vi "Create Job VI from Template.vi"() -> ()   [LabVIEW 2013]
uses:
  JobCreatorData -- cluster.ctl
panel:
  in  "Cron Job Templates":i32(listbox)
  in  "Instantiate Job":bool
  # "Select a Cron Job Template for instantiation"
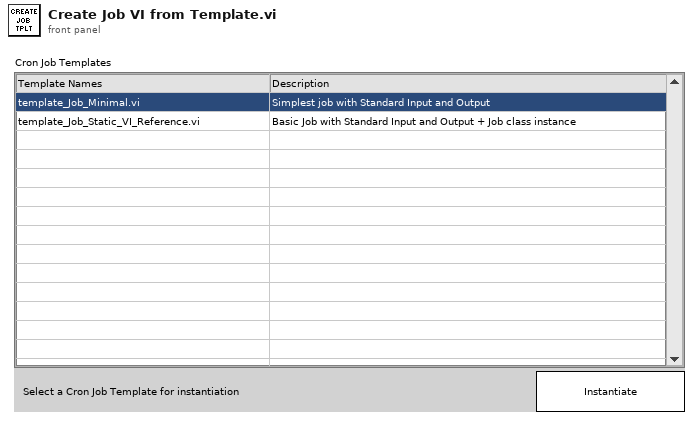
[diagram p1: front panel]
types:
  T1 = enum16{"Initialize", "Discover Template", "Idle", "Create Template", "Exit"}
  T2 = cluster{"App Instance":refnum<vi>, "Active Project":refnum<vi>, "templates":variant, "Cron Folder":path}
  T3 = enum8{"Enabled", "Disabled", "Disabled and Grayed Out"}
  T4 = typedef "JobCreatorData -- cluster.ctl" = cluster{"Path":path, "Name":string, "Description":string}
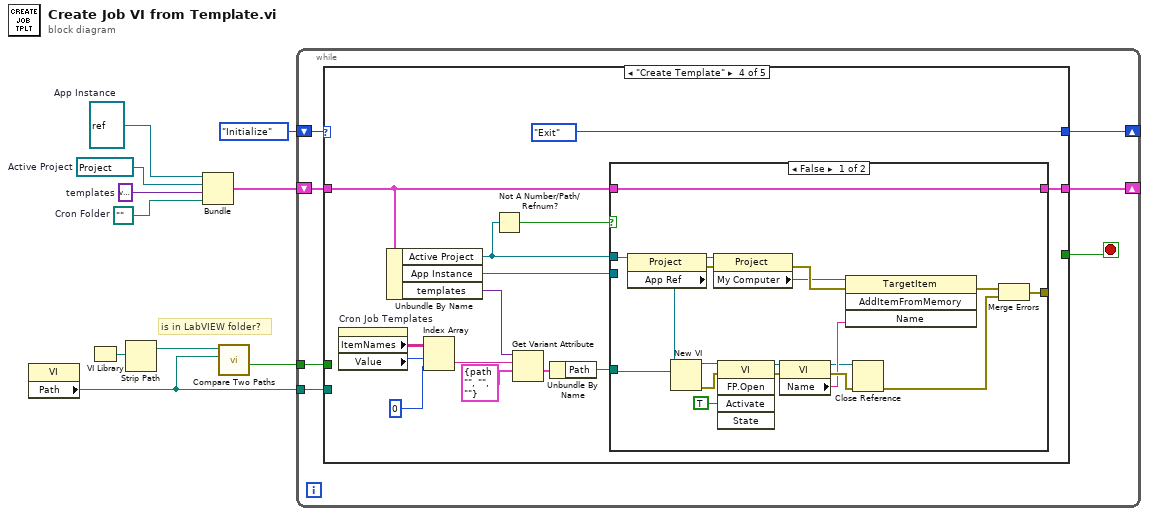
[diagram p0: block diagram]
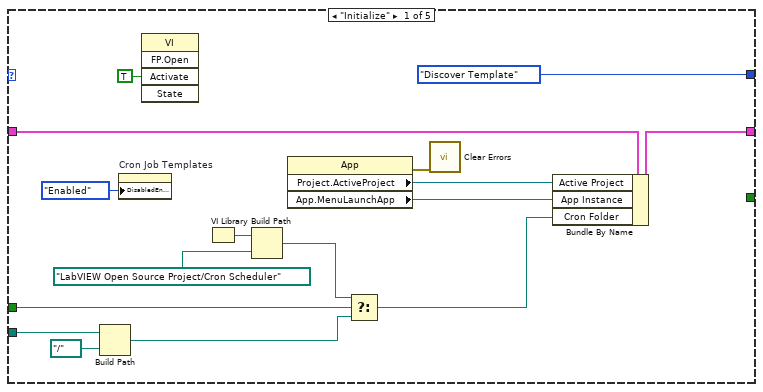
[diagram p2: hidden frame]
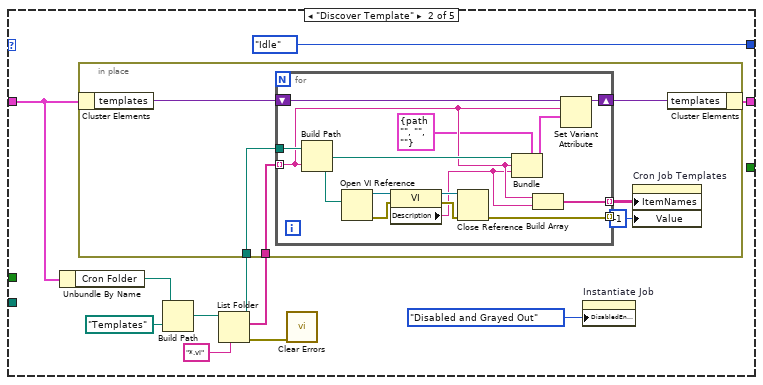
[diagram p3: hidden frame]
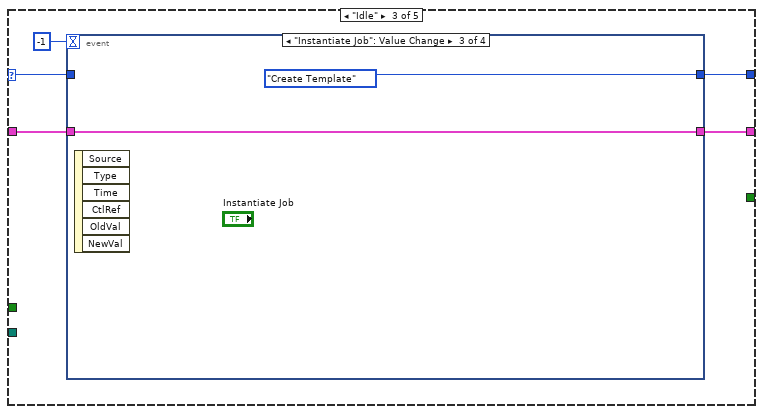
[diagram p4: hidden frame]
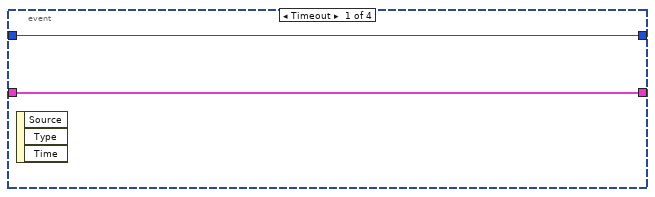
[diagram p5: hidden frame]
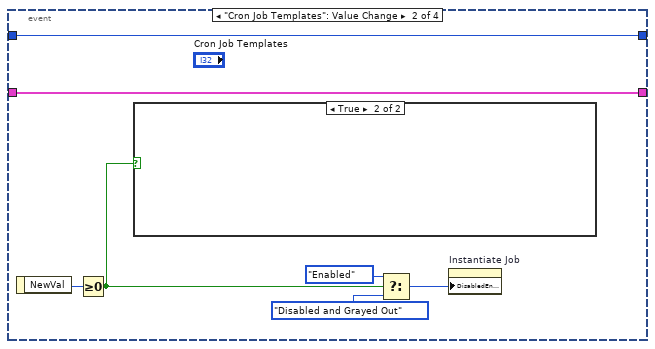
[diagram p6: hidden frame]
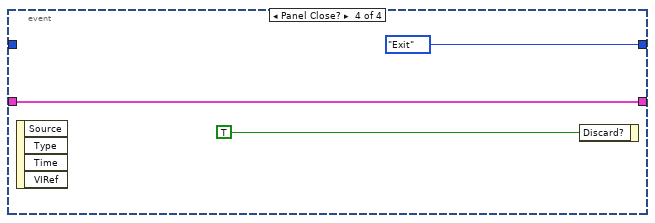
[diagram p8: hidden frame]
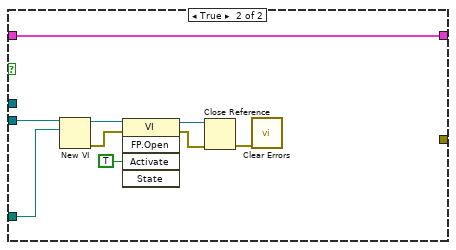
[diagram p9: hidden frame]
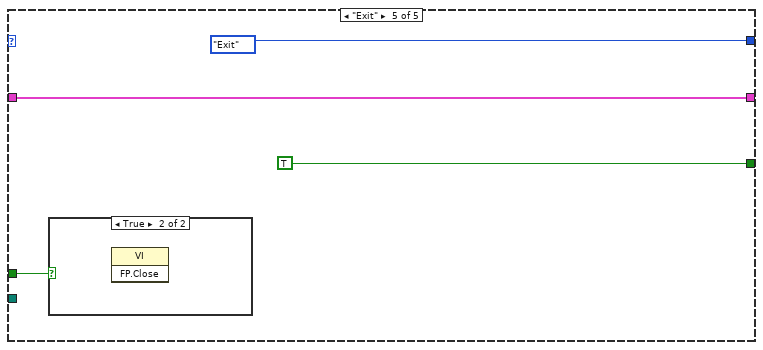
[diagram p10: hidden frame]
diagram:
  w9 = path ""  # Cron Folder
  w8 = variant  # templates
  w7 = refnum<vi> refnum  # App Instance
  w5 = refnum<vi> refnum  # Active Project
  # "is in LabVIEW folder?"
  n1 = property class="VI"() -> ("Path"=w2:path)  [unwired: 2 in, 2 out]
  n2 = VI Library() -> (path=w3:path)
  n3 = Strip Path(path=w3) -> (stripped path=w4:path)  [unwired: 1 out]
  n4 = Bundle("App Instance"=w7, "Active Project"=w5, "templates"=w8, "Cron Folder"=w9) -> (w6:T2)  [unwired: 1 in]
  n5 = call <vilib>:"Compare Two Paths.vi"("Path 2"=w2, "Path 1"=w4) -> ("Path 2 Relative to Path 1?"=w1:bool)  [unwired: 6 in, 3 out]
  n6 = while {
    shift-right: [w16] -> _
    shift-left: T1."Initialize" -> [w17]
    shift-right: [w14] -> _
    shift-left: w6 -> [w15]
    tunnel: w2 -> [w12]
    tunnel: w1 -> [w11]
    stop <- w13 stop-if-true
    n7 = case shown="\"Create Template\"" w17 {
      selector: w17 -> [_ _ w65 _ _]
      tunnel: [T1."Discover Template" T1."Idle" w68 T1."Exit" T1."Exit"] -> w16
      tunnel: w15 -> [w31 w41 w67 w88 w128]
      tunnel: [w32 w43 w66 w87 w128] -> w14
      tunnel: [_ _ _ _ TRUE] -> w13
      tunnel: w12 -> [w19 _ _ _ _]
      tunnel: w11 -> [w18 _ _ _ w126]
      frame "Initialize" {
        n8 = Build Path(base path=w19, name or relative path=path "../.." ("VI Path")) -> (appended path=w27:path)
        n9 = property on="Cron Job Templates" class="MCListbox (strict)"("DisabledEnum"=T3."Enabled" ("Disabled")) -> ()  [unwired: 2 in, 2 out]
        n10 = invoke class="VI" method="FP.Open"("Activate"=TRUE ("Activate?")) -> ()  [unwired: 4 in, 5 out]
        n11 = VI Library() -> (path=w20:path)
        n12 = Build Path(base path=w20, name or relative path=path "LabVIEW Open Source Project/Cron Scheduler" ("VI Path")) -> (appended path=w23:path)
        n13 = property class="App"() -> (error out=w30:errorcluster, "Project.ActiveProject"=w26:refnum<vi>, "App.MenuLaunchApp"=w29:refnum<vi>)  [unwired: 2 in, 1 out]
        n14 = Select(t=w23, s=w18, f=w27) -> (s? t:f=w24:path)
        n15 = call <vilib>:"Clear Errors.vi"("error in (no error)"=w30) -> ()  [unwired: 6 in, 1 out]
        n16 = Bundle By Name(cluster=w31, "Active Project"=w26, "App Instance"=w29, "Cron Folder"=w24) -> (w32:T2)
      }
      frame "Discover Template" {
        n17 = Unbundle By Name(w41) -> ("Cron Folder"=w40:path)
        n18 = Build Path(base path=w40, name or relative path=path "Templates" ("VI Path")) -> (appended path=w39:path)
        n19 = List Folder(path=w39, pattern="*.vi") -> (path out=w36:path, filenames=w37:string[], error out=w35:errorcluster)  [unwired: 2 in, 1 out]
        n20 = in-place {
          in-place-border: w37 -> [w48]
          in-place-border: w36 -> [w47]
          n21 = in-place-cluster #1(w41) -> ("templates"=w50:variant)
          n22 = for {
            tunnel: w48 -> [w54] mode=indexing
            tunnel: w47 -> [w62]
            tunnel: [w57] -> _ mode=indexing
            tunnel: [w52] -> w46 mode=indexing
            shift-right: [w63] -> w49
            shift-left: w50 -> [w64]
            n23 = Build Path(base path=w62, name or relative path=w54) -> (appended path=w60:path)
            n24 = Open VI Reference(vi path=w60) -> (vi reference=w59:refnum<vi>, error out=w56:errorcluster)  [unwired: 5 in]
            n25 = property class="VI"(reference=w59, error in=w56) -> (reference out=w58:refnum<vi>, error out=w55:errorcluster, "Description"=w53:string)
            n26 = Close Reference(reference=w58, error in (no error)=w55) -> (error out=w57:errorcluster)
            n27 = Bundle(cluster=T4 {"Path"=path "", "Name"="", "Description"=""} ("Job Creator Data"), "Path"=w60, "Name"=w54, "Description"=w53) -> (w61:T4)
            n28 = Build Array(w54, w53) -> (w52:string[])
            n29 = Set Variant Attribute(Variant=w64, name=w54, value=w61) -> (Variant out=w63:variant)  [unwired: 1 in, 2 out]
          }
          n30 = property on="Cron Job Templates" class="MCListbox (strict)"("ItemNames"=w46, "Value"=-1 ("Cron Job Templates")) -> ()  [unwired: 2 in, 2 out]
          n31 = in-place-cluster #1("templates"=w49) -> (w43:T2)
        }
        n32 = call <vilib>:"Clear Errors.vi"("error in (no error)"=w35) -> ()  [unwired: 6 in, 1 out]
        n33 = property on="Instantiate Job" class="Bool"("DisabledEnum"=T3."Disabled and Grayed Out" ("Disabled")) -> ()  [unwired: 2 in, 2 out]
      }
      frame "Idle" {
        n34 = event shown="[2] \"Instantiate Job\": Value Change" {
          selector: _ -> [_ _ _ _]
          dyn-events: _ -> [_ _ _ _]
          timeout: -1 -> [_ _ _ _]
          tunnel: [w70 w72 T1."Create Template" T1."Exit"] -> w68
          tunnel: w67 -> [w71 w78 w80 w81]
          tunnel: [w71 w78 w80 w81] -> w66
          tunnel: w65 -> [w70 w72 _ _]
          event Timeout {
            n35 = event-data() -> ()  [unwired: 1 in, 3 out]
          }
          event "Cron Job Templates": Value Change {
            n36 = event-data() -> ("NewVal"=w77:i32)  [unwired: 1 in]
            n37 = Greater Or Equal To 0?(x=w77) -> (x >= 0?=w73:bool)
            n38 = case shown="True" w73 {
              frame False {
              }
              frame True {
              }
            }
            n39 = Select(t=T3."Enabled" ("Disabled"), s=w73, f=T3."Disabled and Grayed Out" ("Disabled")) -> (s? t:f=w74:T3)
            n40 = property on="Instantiate Job" class="Bool"("DisabledEnum"=w74) -> ()  [unwired: 2 in, 2 out]
          }
          event "Instantiate Job": Value Change {
            n41 = event-data() -> ()  [unwired: 1 in, 6 out]
          }
          event Panel Close? {
            n42 = event-data() -> ()  [unwired: 1 in, 4 out]
            n43 = event-data("Discard?"=TRUE) -> ()  [unwired: 1 in, 1 out]
          }
        }
      }
      frame "Create Template" {
        n44 = property on="Cron Job Templates" class="MCListbox (strict)"() -> ("ItemNames"=w96:string[][], "Value"=w94:i32)  [unwired: 2 in, 2 out]
        n45 = Unbundle By Name(w88) -> ("Active Project"=w84:refnum<vi>, "App Instance"=w85:refnum<vi>, "templates"=w92:variant)
        n46 = Index Array(array=w96, index (row)=w94, index (col)=0 ("disabled index (col)")) -> (element=w93:string)
        n47 = Not A Number/Path/Refnum?(number/path/refnum=w84) -> (NaN/Path/Refnum?=w89:bool)
        n48 = Get Variant Attribute(Variant=w92, name=w93, default value (empty Variant)=T4 {"Path"=path "", "Name"="", "Description"=""}) -> (value=w90:T4)  [unwired: 1 in, 3 out]
        n49 = Unbundle By Name(w90) -> ("Path"=w86:path)
        n50 = case shown="False" w89 {
          tunnel: w88 -> [w116 w125]
          tunnel: [w116 w125] -> w87
          tunnel: w86 -> [w98 w118]
          tunnel: w85 -> [_ w119]
          tunnel: w84 -> [w100 _]
          tunnel: [w99 _] -> _
          frame False {
            n51 = property class="Project"(reference=w100) -> (reference out=w104:refnum<vi>, error out=w107:errorcluster, "App Ref"=w103:refnum<vi>)  [unwired: 1 in]
            n52 = New VI(10:w98, 11:w103) -> (0:w110:errorcluster, 3:w102:refnum<vi>)  [unwired: 5 in]
            n53 = property class="Project"(reference=w104, error in=w107) -> (error out=w113:errorcluster, "My Computer"=w105:refnum<vi>)  [unwired: 1 out]
            n54 = invoke class="VI" method="FP.Open"(reference=w102, error in=w110, "Activate"=TRUE ("Activate?")) -> (reference out=w106:refnum<vi>, error out=w111:errorcluster)  [unwired: 2 in, 3 out]
            n55 = property class="VI"(reference=w106, error in=w111) -> (reference out=w108:refnum<vi>, error out=w112:errorcluster, "Name"=w109:string)
            n56 = invoke class="TargetItem" method="AddItemFromMemory"(reference=w105, error in=w113, "Name"=w109) -> (error out=w114:errorcluster)  [unwired: 1 in, 3 out]
            n57 = Close Reference(reference=w108, error in (no error)=w112) -> (error out=w115:errorcluster)
            n58 = Merge Errors(w114, w115) -> (w99:errorcluster)
          }
          frame True {
            n59 = New VI(10:w118, 11:w119) -> (0:w123:errorcluster, 3:w121:refnum<vi>)  [unwired: 5 in]
            n60 = invoke class="VI" method="FP.Open"(reference=w121, error in=w123, "Activate"=TRUE ("Activate?")) -> (reference out=w122:refnum<vi>, error out=w124:errorcluster)  [unwired: 2 in, 3 out]
            n61 = Close Reference(reference=w122, error in (no error)=w124) -> (error out=w117:errorcluster)
            n62 = call <vilib>:"Clear Errors.vi"("error in (no error)"=w117) -> ()  [unwired: 6 in, 1 out]
          }
        }
      }
      frame "Exit" {
        n63 = case shown="True" w126 {
          frame False {
          }
          frame True {
            n64 = invoke class="VI" method="FP.Close"() -> ()  [unwired: 3 in, 3 out]
          }
        }
      }
    }
  }
